vi "Trigger Core Instance.vi"(8 "error in (no error)":errorcluster, 11 "CaptureDetectionLoopDataIn":T1={"Period"=-1, "Reset"=TRUE, "Iteration"=0, "Capture"=path "", "Mode"={"Replay"=enum."None", "Record"=enum."None"}, "Replay Run ID"="", "Frame Number"=0, "Core Module ID"=0, "EventRecorderLaunched"=FALSE, "Frame 0 relative seconds"=0.0} {"Frame 0 relative seconds" format="%_19f"}) -> (0 "error out":errorcluster, 3 "CaptureDetectionLoopDataOut":T1={"Period"=-1, "Reset"=TRUE, "Iteration"=0, "Capture"=path "", "Mode"={"Replay"=enum."None", "Record"=enum."None"}, "Replay Run ID"="", "Frame Number"=0, "Core Module ID"=0, "EventRecorderLaunched"=FALSE, "Frame 0 relative seconds"=0.0} {"Frame 0 relative seconds" format="%_19f"})   [LabVIEW 2026, in "Launcher.lvlib"]
uses:
  Launcher.lvlib
  Capture detection loop data--cluster.ctl
  Mode.ctl
  ReplayMode.ctl
  RecordMode.ctl
  <userlib>/_OpenG.lib/boolean/boolean.llb/openg_boolean__ogtk.lvlib
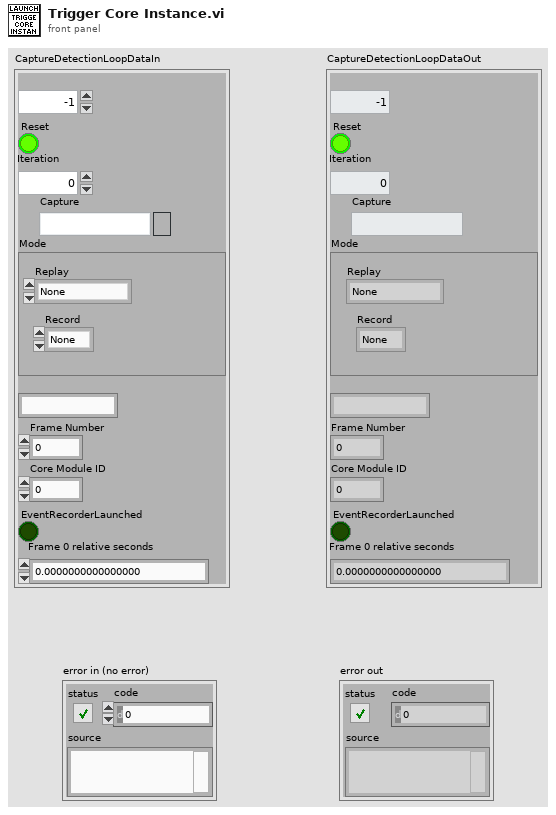
[diagram p1: front panel]
types:
  T1 = typedef "Capture detection loop data--cluster.ctl" = cluster{"Period":i32, "Reset":bool, "Iteration":i32, "Capture":path, "Mode":T2, "Replay Run ID":string, "Frame Number":u32, "Core Module ID":i32, "EventRecorderLaunched":bool, "Frame 0 relative seconds":dbl}
  T2 = typedef "Mode.ctl" = cluster{"Replay":T3, "Record":T4}
  T3 = typedef "ReplayMode.ctl" = enum16{"None", "User Events"}
  T4 = typedef "RecordMode.ctl" = enum16{"None", "User Events", "Benchmarks", "User Events and Benchmarks"}
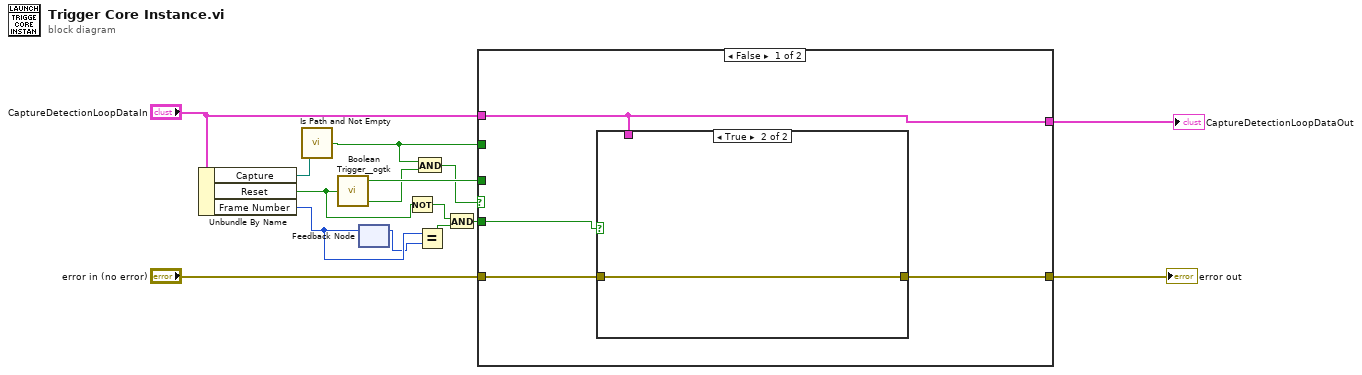
[diagram p0: block diagram]
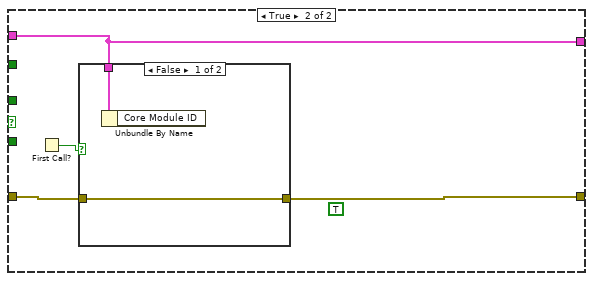
[diagram p3: hidden frame]
diagram:
  n1 = Unbundle By Name("CaptureDetectionLoopDataIn") -> ("Capture"=w10:path, "Reset"=w2:bool, "Frame Number"=w6:u32)
  n2 = call <vilib>:"Is Path and Not Empty.vi"("path"=w10) -> ("Is Path and Not Empty?"=w9:bool)  [unwired: 4 in]
  n3 = call <userlib>:"Boolean Trigger__ogtk.vi"("Boolean Input"=w2) -> ("Rising Edge"=w13:bool, "Falling Edge"=w7:bool)  [unwired: 1 in]
  n4 = feedback-in #1(w6) -> ()
  n5 = feedback #1() -> (w5:u32)  [unwired: 1 in]
  n6 = Not(x=w2) -> (.not. x?=w1:bool)
  n7 = And(x=w9, y=w7) -> (x .and. y?=w8:bool)
  n8 = Equal?(x=w6, y=w5) -> (x = y?=w4:bool)
  n9 = And(x=w1, y=w4) -> (x .and. y?=w3:bool)
  n10 = case shown="False" w8 {
    tunnel: "error in (no error)" -> [w19 w25]
    tunnel: [w18 w22] -> w14
    tunnel: w13 -> [_ _]
    tunnel: "CaptureDetectionLoopDataIn" -> [w17 w24]
    tunnel: [w17 w24] -> w11
    tunnel: w9 -> [_ _]
    tunnel: w3 -> [w16 _]
    frame False {
      n11 = case shown="True" w16 {
        tunnel: w19 -> [w20 w21]
        tunnel: [w20 w21] -> w18
        tunnel: w17 -> [_ _]
        frame False {
        }
        frame True {
        }
      }
    }
    frame True {
      (unwired) TRUE ("Show Main VI Diagram on Init (F)")
      n12 = First Call?() -> (First Call?: T/F=w23:bool)
      n13 = case shown="False" w23 {
        tunnel: w25 -> [w26 w28]
        tunnel: [w26 w28] -> w22
        tunnel: w24 -> [w27 _]
        frame False {
          n14 = Unbundle By Name(w27) -> ()  [unwired: 1 out]
        }
        frame True {
        }
      }
    }
  }
  "CaptureDetectionLoopDataOut" <- w11
  "error out" <- w14
